vi "Write Lines.vi"(8 "error in (no error)":errorcluster, 10 "Lines":T1[](array[typedef]), 11 "Shared Memory configuration in":refnum<class "Shared Memory configuration.lvclass">) -> (0 "error out":errorcluster, 3 "Shared Memory configuration out":refnum<class "Shared Memory configuration.lvclass">)   [LabVIEW 2014, in "Shared Memory configuration.lvclass"]
uses:
  Shared Memory configuration.lvclass
  Line.ctl
  <vilib>/NI/Tag Bus Module Framework/channel/TBM channel.lvclass
  Shared Memory configuration.lvclass/Shared Memory configuration.ctl
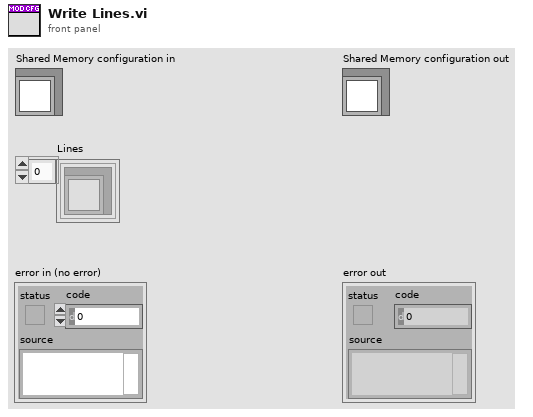
[diagram p1: front panel]
types:
  T1 = typedef "Shared Memory configuration.lvclass/Line.ctl" = cluster{"channel":refnum<class "TBM channel.lvclass">}
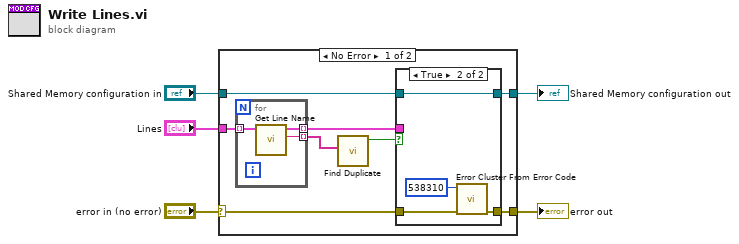
[diagram p0: block diagram]
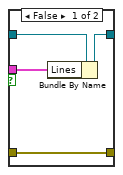
[diagram p2: hidden frame]
diagram:
  n1 = case shown="No Error" "error in (no error)" {
    selector: "error in (no error)" -> [w8 w25]
    tunnel: [w7 w25] -> w4
    tunnel: [w10 w26] -> w2
    tunnel: "Shared Memory configuration in" -> [w13 w26]
    tunnel: "Lines" -> [w12 _]
    frame No Error {
      n2 = for {
        tunnel: w12 -> [w24] mode=indexing
        tunnel: [w23] -> w6 mode=indexing
        tunnel: [w22] -> w11 mode=indexing
        n3 = call "Get Line Name.vi"("Line in"=w24) -> ("Name"=w22:string, "Line out"=w23:T1)  [unwired: 8 in, 1 out]
      }
      n4 = call "Find Duplicate.vi"("Array"=w11) -> ("Duplicate"=w9:bool)  [unwired: 8 in, 2 out]
      n5 = case shown="True" w9 {
        tunnel: w13 -> [w17 w18]
        tunnel: [w16 w18] -> w10
        tunnel: w8 -> [w15 w20]
        tunnel: [w15 w19] -> w7
        tunnel: w6 -> [w14 _]
        frame False {
          n6 = Bundle By Name(cluster=w17, "Lines"=w14) -> (w16:refnum<class "Shared Memory configuration.lvclass">)
        }
        frame True {
          n7 = call <vilib>:"Error Cluster From Error Code.vi"("error in (no error)"=w20, "error code (0)"=538310) -> ("error out"=w19:errorcluster)  [unwired: 7 in]
        }
      }
    }
    frame Error {
    }
  }
  "error out" <- w4
  "Shared Memory configuration out" <- w2
